vi "Send API Request v4.vi"(5 "AWS Core":refnum<class "HTTP Request.lvclass">, 6 "request body":string, 7 "Authorization":string, 8 "error in (no error)":errorcluster, 9 "HTTP-Verb":string, 10 "Host String":string, 11 "Client Handle":T1) -> (0 "error out":errorcluster, 1 "Call Result":string, 2 "response body":string, 3 "response headers":string, 4 "Redirect endpoint":string)   [LabVIEW 2015, in "NI_AWS_Core.lvlib" / "HTTP Request.lvclass"]
uses:
  HTTP Request.lvclass
  <vilib>/httpClient/ClientHandle.ctl
  <vilib>/httpClient/PUTBuffer.vi
  <vilib>/httpClient/POSTBuffer.vi
  <vilib>/httpClient/LabVIEWHTTPClient.lvlib
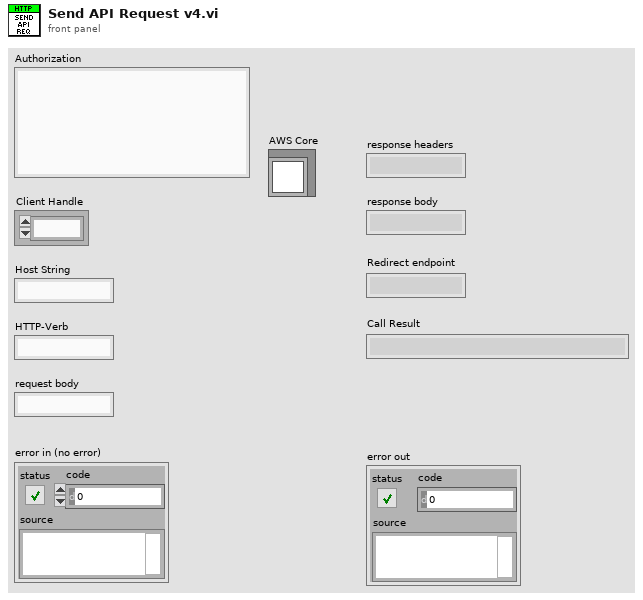
[diagram p1: front panel]
types:
  T1 = typedef "LabVIEWHTTPClient.lvlib/ClientHandle.ctl" = refnum<k1>
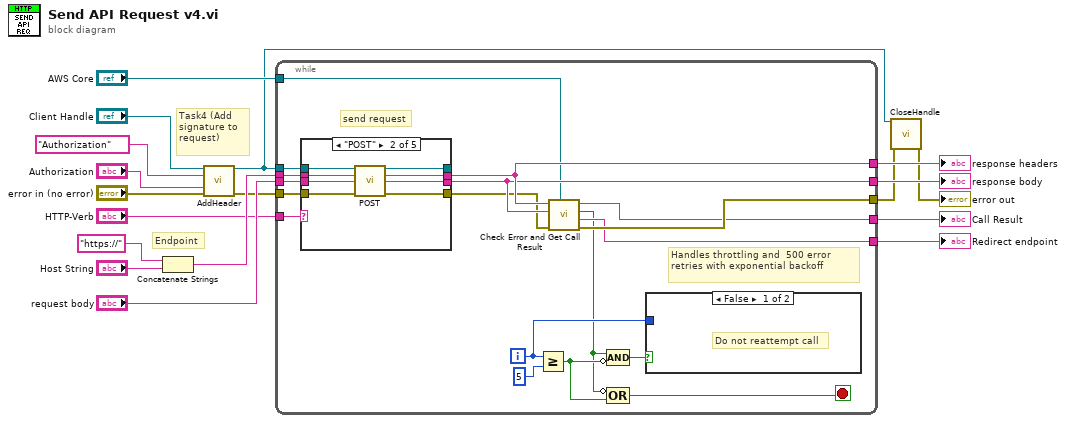
[diagram p0: block diagram]
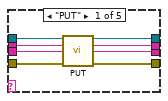
[diagram p2: hidden frame]
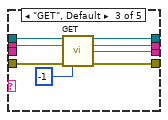
[diagram p3: hidden frame]
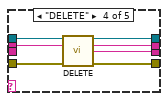
[diagram p4: hidden frame]
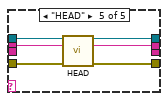
[diagram p5: hidden frame]
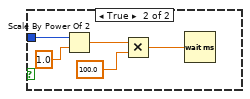
[diagram p6: hidden frame]
diagram:
  # "Endpoint"
  # "Task4 (Add signature to request)"
  n1 = Concatenate Strings("https://" ("string"), "Host String") -> (w17:string)
  n2 = call <vilib>:"AddHeader.vi"("client handle"="Client Handle", "header"="Authorization", "value"="Authorization", "error in (no error)"="error in (no error)") -> ("client handle out"=w1:T1, "error out"=w14:errorcluster)  [unwired: 10 in]
  n3 = while {
    tunnel: w1 -> [w33]
    tunnel: [w21] -> w5
    tunnel: w17 -> [w35]
    tunnel: [w26] -> w8
    tunnel: "request body" -> [w36]
    tunnel: [w25] -> w7
    tunnel: "HTTP-Verb" -> [w32]
    tunnel: [w23] -> w6
    tunnel: w14 -> [w34]
    tunnel: [w31] -> w2
    tunnel: "AWS Core" -> [w20]
    i -> [w30]
    stop <- w29 stop-if-true
    # "Handles throttling and  500 error retries with exponential backoff"
    # "send request"
    n4 = case shown="\"POST\"" w32 {
      tunnel: [w39 w52 w59 w62 _] -> w25
      tunnel: [w38 w51 w60 w61 w73] -> w26
      tunnel: w35 -> [w43 w50 w56 w65 w71]
      tunnel: w33 -> [w44 w49 w55 w64 w69]
      tunnel: w36 -> [w42 w48 _ _ _]
      tunnel: w34 -> [w41 w47 w57 w66 w70]
      tunnel: [w40 w46 w58 w67 w72] -> w19
      tunnel: [w37 w45 w54 w63 w68] -> _
      frame "PUT" {
        n5 = call-poly <vilib>:"PUT.vi"("client handle"=w44, "url"=w43, "buffer"=w42, "error in (no error)"=w41) -> ("client handle out"=w37:T1, "headers"=w38:string, "body"=w39:string, "error out"=w40:errorcluster)  [unwired: 8 in]
      }
      frame "POST" {
        n6 = call-poly <vilib>:"POST.vi"("client handle"=w49, "url"=w50, "buffer"=w48, "error in (no error)"=w47) -> ("client handle out"=w45:T1, "headers"=w51:string, "body"=w52:string, "error out"=w46:errorcluster)  [unwired: 8 in]
      }
      frame "GET", Default {
        n7 = call <vilib>:"GET.vi"("client handle"=w55, "url"=w56, "error in (no error)"=w57, "timeout (10000)"=-1) -> ("client handle out"=w54:T1, "headers"=w60:string, "body"=w59:string, "error out"=w58:errorcluster)  [unwired: 8 in]
      }
      frame "DELETE" {
        n8 = call <vilib>:"DELETE.vi"("client handle"=w64, "url"=w65, "error in (no error)"=w66) -> ("client handle out"=w63:T1, "headers"=w61:string, "body"=w62:string, "error out"=w67:errorcluster)  [unwired: 9 in]
      }
      frame "HEAD" {
        n9 = call <vilib>:"HEAD.vi"("client handle"=w69, "url"=w71, "error in (no error)"=w70) -> ("client handle out"=w68:T1, "headers"=w73:string, "error out"=w72:errorcluster)  [unwired: 10 in]
      }
    }
    n10 = Greater Or Equal?(x=w30, y=5) -> (x >= y?=w27:bool)
    n11 = call "Check Error and Get Call Result.vi"("AWS Core"=w20, "error in (no error)"=w19, "Response body"=w25, "Response header"=w26) -> ("error out"=w31:errorcluster, "Redirect endpoint"=w23:string, "500 Or Throttled?"=w22:bool, "Call Result"=w21:string)  [unwired: 4 in]
    n12 = Compound Arithmetic op=AND(w22, invert w27) -> (w28:bool)
    n13 = Compound Arithmetic op=OR(invert w22, w27) -> (w29:bool)
    n14 = case shown="False" w28 {
      tunnel: w30 -> [_ w77]
      frame False {
        # "Do not reattempt call"
      }
      frame True {
        n15 = Scale By Power Of 2(n=w77, x=1.0) -> (x*2^n=w75:dbl)
        n16 = Multiply(x=w75, y=100.0) -> (x*y=w76:dbl)
        n17 = Wait (ms)(milliseconds to wait=w76) -> ()  [unwired: 1 out]
      }
    }
  }
  "response headers" <- w8
  "response body" <- w7
  "Redirect endpoint" <- w6
  "Call Result" <- w5
  n18 = call <vilib>:"CloseHandle.vi"("client handle"=w1, "error in (no error)"=w2) -> ("error out"=→"error out":errorcluster)  [unwired: 13 in]
